vi "Game_Start.vi"(0 "Context":T1={"Screen"=enum."Settings", "Settings"=[0, 0, 1, 1], "Board"={"Grid"=array15x15[225 elements], "Move History"=[], "Last Move"={"Row"=-1, "Col"=-1, "Stone"=enum."Empty"}}, "Status"=enum."Idle", "Game ID"=0, "Player Stone"=enum."Black", "Hover"={"Row"=-1, "Col"=-1, "Stone"=enum."Empty"}, "Hover Button"=-1, "Win Line"=[], "Score 1"=0, "Score 2"=0, "Draws"=0, "Status Text"="", "Status Color"=0}, 5 "Reset Scores":bool, 11 "error in":errorcluster) -> (4 "Context out":T1={"Screen"=enum."Settings", "Settings"=[0, 0, 1, 1], "Board"={"Grid"=array15x15[225 elements], "Move History"=[], "Last Move"={"Row"=-1, "Col"=-1, "Stone"=enum."Empty"}}, "Status"=enum."Idle", "Game ID"=0, "Player Stone"=enum."Black", "Hover"={"Row"=-1, "Col"=-1, "Stone"=enum."Empty"}, "Hover Button"=-1, "Win Line"=[], "Score 1"=0, "Score 2"=0, "Draws"=0, "Status Text"="", "Status Color"=0}, 6 "Need AI":bool, 15 "error out":errorcluster)   [LabVIEW 2026]
doc: "새 판 시작: 바둑판 초기화, Game ID 증가, 게임 화면으로 전환. Reset Scores면 점수도 0.\nNeed AI = AI 대전에서 플레이어가 백이라 AI가 먼저 둘 때 True."
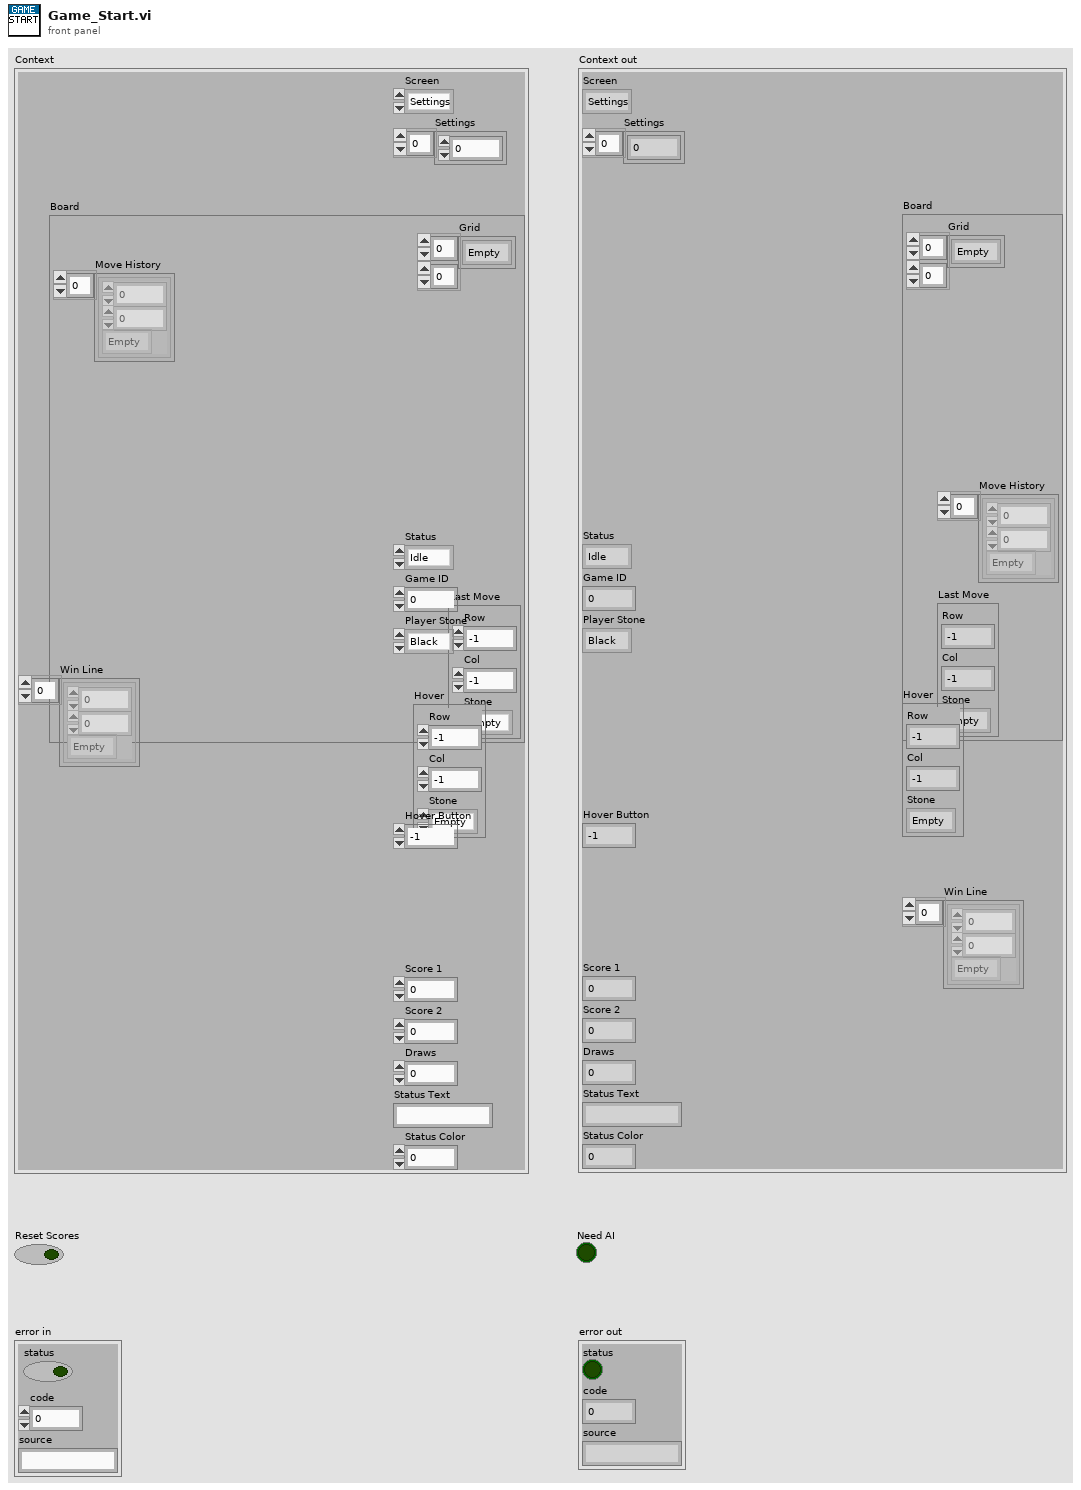
[diagram p1: front panel]
types:
  T1 = cluster{"Screen":enum16{"Settings", "Game"}, "Settings":i32[], "Board":cluster{"Grid":enum8{"Empty", "Black", "White"}[][], "Move History":cluster{"Row":i32, "Col":i32, "Stone":enum8{"Empty", "Black", "White"}}[], "Last Move":cluster{"Row":i32, "Col":i32, "Stone":enum8{"Empty", "Black", "White"}}}, "Status":enum16{"Idle", "Player Turn", "AI Thinking", "Game Over"}, "Game ID":u32, "Player Stone":enum8{"Empty", "Black", "White"}, "Hover":cluster{"Row":i32, "Col":i32, "Stone":enum8{"Empty", "Black", "White"}}, "Hover Button":i32, "Win Line":cluster{"Row":i32, "Col":i32, "Stone":enum8{"Empty", "Black", "White"}}[], "Score 1":i32, "Score 2":i32, "Draws":i32, "Status Text":string, "Status Color":u32}
  T2 = cluster{"Row":i32, "Col":i32, "Stone":enum8{"Empty", "Black", "White"}}[]
  T3 = cluster{"Row":i32, "Col":i32, "Stone":enum8{"Empty", "Black", "White"}}
  T4 = cluster{"Grid":enum8{"Empty", "Black", "White"}[][], "Move History":cluster{"Row":i32, "Col":i32, "Stone":enum8{"Empty", "Black", "White"}}[], "Last Move":cluster{"Row":i32, "Col":i32, "Stone":enum8{"Empty", "Black", "White"}}}
  T5 = enum16{"Idle", "Player Turn", "AI Thinking", "Game Over"}
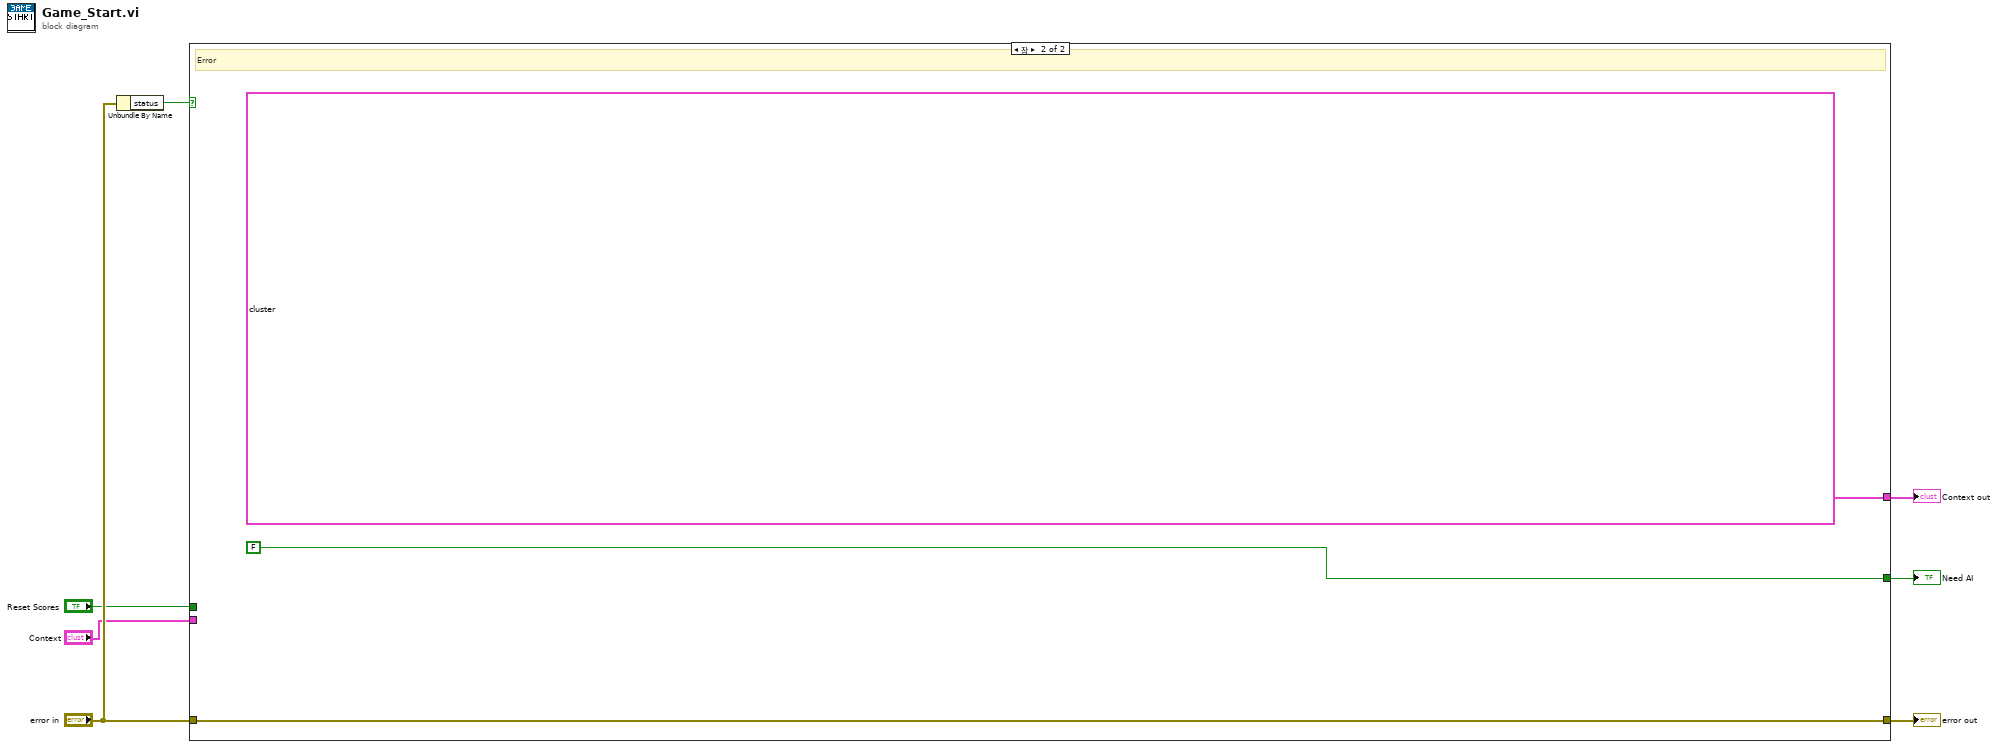
[diagram p0: block diagram]
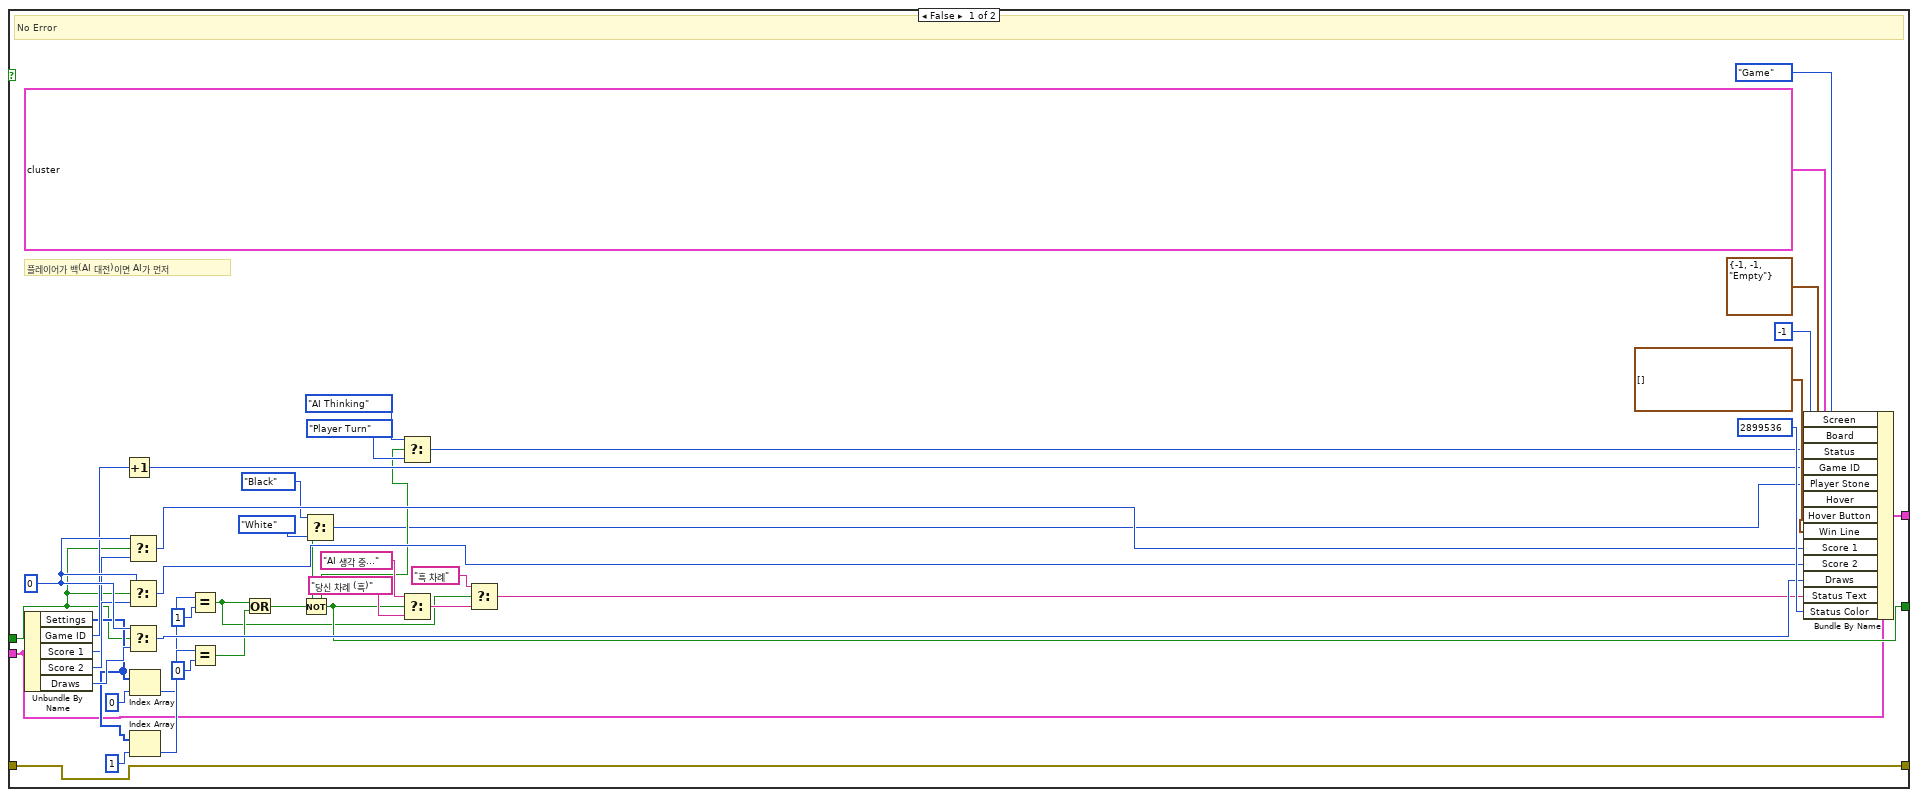
[diagram p2: hidden frame]
diagram:
  n1 = Unbundle By Name("error in") -> ("status"=w4:bool)
  n2 = case shown="참" w4 {
    tunnel: "Context" -> [w8 _]
    tunnel: "Reset Scores" -> [w9 _]
    tunnel: "error in" -> [w10 w49]
    tunnel: [w10 w49] -> w7
    tunnel: [w28 FALSE] -> w6
    tunnel: [w48 T1 {"Screen"=enum."Settings", "Settings"=[0, 0, 1, 1], "Board"={"Grid"=array15x15[225 elements], "Move History"=[], "Last Move"={"Row"=-1, "Col"=-1, "Stone"=enum."Empty"}}, "Status"=enum."Idle", "Game ID"=0, "Player Stone"=enum."Black", "Hover"={"Row"=-1, "Col"=-1, "Stone"=enum."Empty"}, "Hover Button"=-1, "Win Line"=[], "Score 1"=0, "Score 2"=0, "Draws"=0, "Status Text"="", "Status Color"=0}] -> w5
    frame False {
      w37 = 0
      # "플레이어가 백(AI 대전)이면 AI가 먼저"
      # "No Error"
      n3 = Unbundle By Name(w8) -> ("Settings"=w11:i32[], "Game ID"=w12:u32, "Score 1"=w13:i32, "Score 2"=w14:i32, "Draws"=w15:i32)
      n4 = Increment(x=w12) -> (x+1=w40:u32)
      n5 = Select(t=w37, s=w9, f=w13) -> (s? t:f=w44:i32)
      n6 = Select(t=w37, s=w9, f=w14) -> (s? t:f=w45:i32)
      n7 = Select(t=w37, s=w9, f=w15) -> (s? t:f=w46:i32)
      n8 = Index Array(array=w11, index=0) -> (element=w17:i32)
      n9 = Index Array(array=w11, index=1) -> (element=w21:i32)
      n10 = Equal?(x=w17, y=1) -> (x = y?=w19:bool)
      n11 = Equal?(x=w21, y=0) -> (x = y?=w23:bool)
      n12 = Or(x=w19, y=w23) -> (x .or. y?=w24:bool)
      n13 = Not(x=w24) -> (.not. x?=w28:bool)
      n14 = Select(t=enum8{"Empty", "Black", "White"}."Black", s=w24, f=enum8{"Empty", "Black", "White"}."White") -> (s? t:f=w27:enum8{"Empty", "Black", "White"})
      n15 = Select(t=T5."AI Thinking", s=w28, f=T5."Player Turn") -> (s? t:f=w31:T5)
      n16 = Select(t="AI 생각 중...", s=w28, f="당신 차례 (흑)") -> (s? t:f=w35:string)
      n17 = Select(t="흑 차례", s=w19, f=w35) -> (s? t:f=w36:string)
      n18 = Bundle By Name(cluster=w8, "Screen"=enum16{"Settings", "Game"}."Game", "Board"=T4 {"Grid"=array15x15[225 elements], "Move History"=[], "Last Move"={"Row"=-1, "Col"=-1, "Stone"=enum."Empty"}}, "Status"=w31, "Game ID"=w40, "Player Stone"=w27, "Hover"=T3 {"Row"=-1, "Col"=-1, "Stone"=enum."Empty"}, "Hover Button"=-1, "Win Line"=T2 [], "Score 1"=w44, "Score 2"=w45, "Draws"=w46, "Status Text"=w36, "Status Color"=u32 2899536) -> (w48:T1)
    }
    frame True {
      # "Error"
    }
  }
  "Context out" <- w5
  "Need AI" <- w6
  "error out" <- w7
